vi "FindMutationByVerIndex.vi"(6 "SerializedClassName":string, 7 "default object":refnum<class "BlueSerializable.lvclass">, 8 "error in (no error)":errorcluster, 9 "Old Name Index":u8, 10 "Library Version":T3, 11 "Mutation History":T4 {"LabVIEW Version" format="%.0x"}) -> (0 "error out":errorcluster, 1 "BlueSerializableVersion":T1, 2 "Mutation Record":T2 {"LabVIEW Version" format="%.0x"})   [LabVIEW 2020, in "BlueSerialization.lvlib" / "BlueSerializer.lvclass"]
uses:
  BlueSerializer.lvclass
  <vilib>/Utility/EditLVLibs/LVClass/Mutation History.ctl
  <vilib>/Utility/EditLVLibs/LVClass/Mutation Record.ctl
  <vilib>/Utility/EditLVLibs/LibVersion.ctl
  BlueSerializableVersion.ctl
  BlueSerializable/BlueSerializable.lvclass
  <resource>/Framework/Providers/BlueSerializationProviderShared/UserCommentToVersion.vi
  <vilib>/Utility/error.llb/Error Cluster From Error Code.vi
  <vilib>/ErrorRing/Error Ring.xnode
  BlueSerializer.lvclass/BlueSerializer.ctl
  <resource>/Framework/Providers/BlueSerializationProviderShared/BlueSerializationProviderShared.lvlib
  <vilib>/Utility/EditLVLibs/Edit LVLibs.lvlib
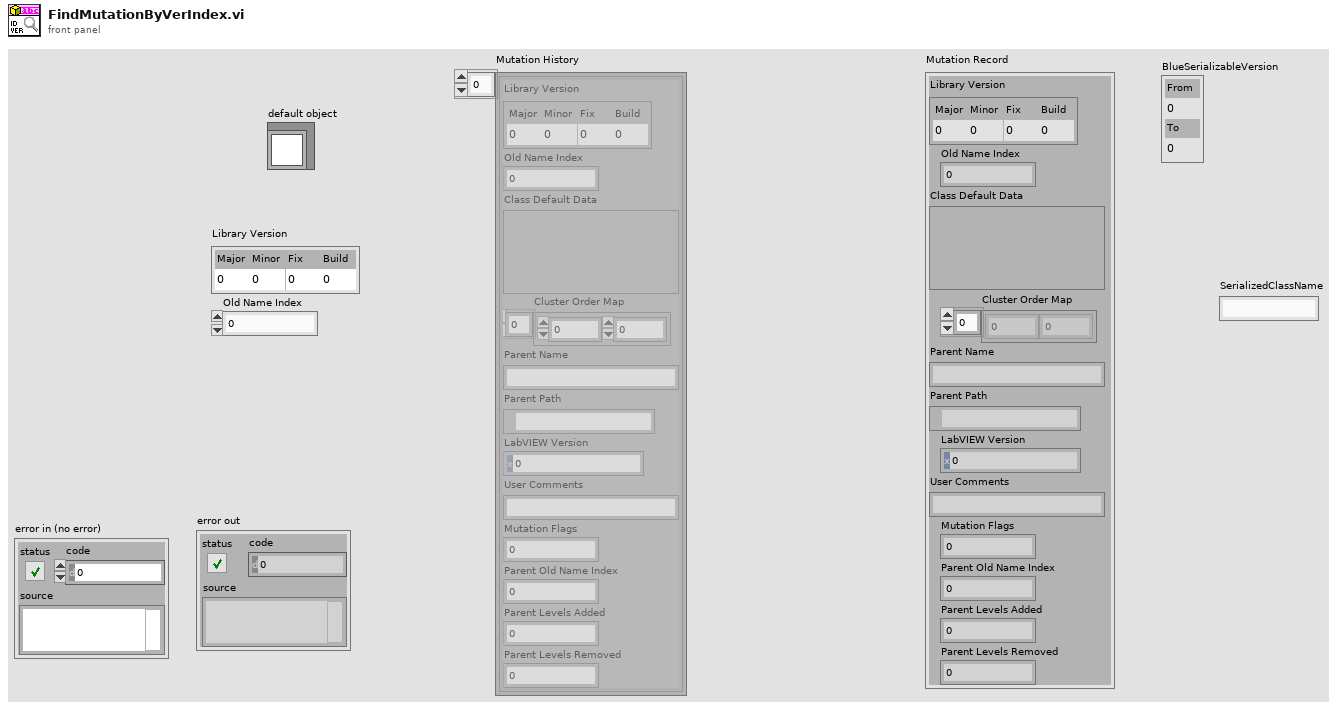
[diagram p1: front panel]
types:
  T1 = typedef "BlueSerialization.lvlib/BlueSerializer.lvclass/BlueSerializableVersion.ctl" = cluster{"From":u16, "To":u16}
  T2 = typedef "Edit LVLibs.lvlib/Mutation Record.ctl" = cluster{"Library Version":T3, "Old Name Index":u8, "Class Default Data":variant, "Cluster Order Map":u32[], "Parent Name":string, "Parent Path":path, "LabVIEW Version":u32, "User Comments":string, "Mutation Flags":u8, "Parent Old Name Index":u8, "Parent Levels Added":u16, "Parent Levels Removed":u16}
  T3 = typedef "Edit LVLibs.lvlib/LibVersion.ctl" = cluster{"Major":u16, "Minor":u16, "Fix":u16, "Build":u16}
  T4 = typedef "Edit LVLibs.lvlib/Mutation History.ctl" = T2[]
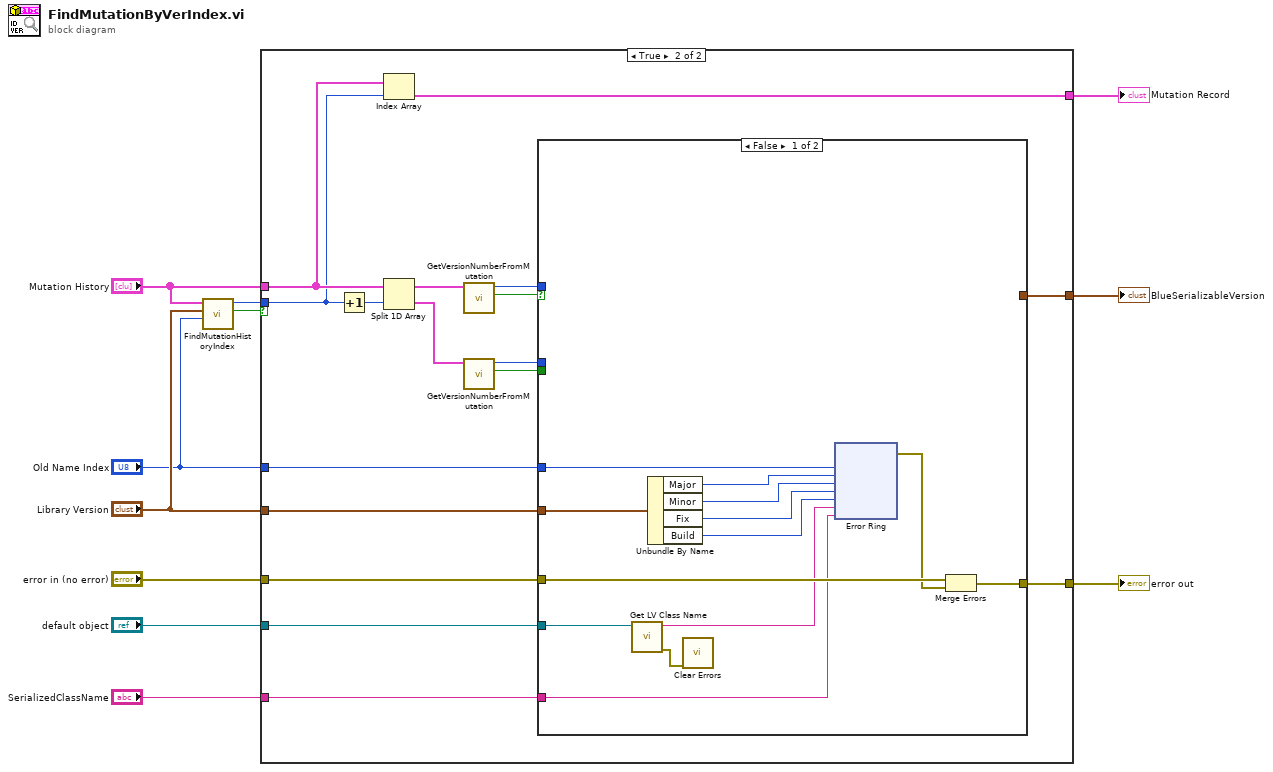
[diagram p0: block diagram]
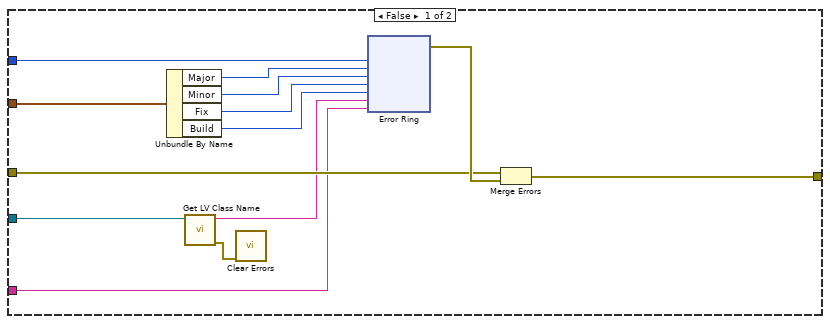
[diagram p2: hidden frame]
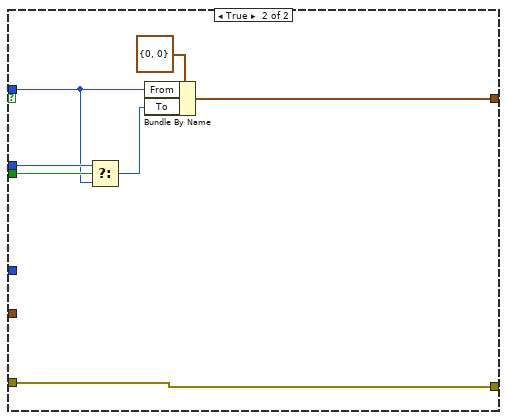
[diagram p3: hidden frame]
diagram:
  n1 = call <resource>:"FindMutationHistoryIndex.vi"("Old Name Index"="Old Name Index", "Library Version"="Library Version", "Mutation History"="Mutation History") -> ("Found?"=w5:bool, "Index"=w6:i32)  [unwired: 7 in]
  n2 = case shown="True" w5 {
    tunnel: "Library Version" -> [w24 w52]
    tunnel: "error in (no error)" -> [w18 w51]
    tunnel: [w17 w50] -> w10
    tunnel: w6 -> [_ w48]
    tunnel: "Mutation History" -> [_ w53]
    tunnel: [_ w54] -> w9
    tunnel: [_ w49] -> w8
    tunnel: "Old Name Index" -> [w16 w40]
    tunnel: "default object" -> [w15 w39]
    tunnel: "SerializedClassName" -> [w12 w38]
    frame False {
      n3 = Unbundle By Name(w24) -> ("Major"=w23:u16, "Minor"=w22:u16, "Fix"=w21:u16, "Build"=w20:u16)
      n4 = call <vilib>:"Get LV Class Name.vi"("object"=w15) -> ("error out"=w13:errorcluster, "class name"=w14:string)  [unwired: 9 in]
      n5 = call <vilib>:"Clear Errors.vi"("error in (no error)"=w13) -> ()  [unwired: 5 in, 2 out]
      n6 = xnode "Error Ring"("parameter 0"=w16, "parameter 1"=w23, "parameter 2"=w22, "parameter 3"=w21, "parameter 4"=w20, "parameter 5"=w14, "parameter 6"=w12) -> ("error out"=w19:errorcluster)
      n7 = Merge Errors(w18, w19) -> (w17:errorcluster)
    }
    frame True {
      n8 = Increment(x=w48) -> (x+1=w47:i32)
      n9 = Index Array(array=w53, index=w48) -> (element=w54:T2)
      n10 = Split 1D Array(array=w53, index=w47) -> (first subarray=w46:T4, second subarray=w41:T4)
      n11 = call <resource>:"GetVersionNumberFromMutation.vi"("Mutation History"=w46) -> ("BlueSerializableVersion found?"=w44:bool, "BlueSerializableVersion"=w45:u16)  [unwired: 9 in]
      n12 = call <resource>:"GetVersionNumberFromMutation.vi"("Mutation History"=w41) -> ("BlueSerializableVersion found?"=w42:bool, "BlueSerializableVersion"=w43:u16)  [unwired: 9 in]
      n13 = case shown="False" w44 {
        tunnel: w42 -> [_ w86]
        tunnel: w45 -> [_ w84]
        tunnel: w43 -> [_ w85]
        tunnel: w52 -> [w63 _]
        tunnel: w51 -> [w62 w82]
        tunnel: [w60 w82] -> w50
        tunnel: [_ w81] -> w49
        tunnel: w40 -> [w59 _]
        tunnel: w39 -> [w57 _]
        tunnel: w38 -> [w55 _]
        frame False {
          n14 = call <vilib>:"Get LV Class Name.vi"("object"=w57) -> ("error out"=w58:errorcluster, "class name"=w56:string)  [unwired: 9 in]
          n15 = Unbundle By Name(w63) -> ("Major"=w67:u16, "Minor"=w66:u16, "Fix"=w65:u16, "Build"=w64:u16)
          n16 = call <vilib>:"Clear Errors.vi"("error in (no error)"=w58) -> ()  [unwired: 5 in, 2 out]
          n17 = xnode "Error Ring"("parameter 0"=w59, "parameter 1"=w67, "parameter 2"=w66, "parameter 3"=w65, "parameter 4"=w64, "parameter 5"=w56, "parameter 6"=w55) -> ("error out"=w61:errorcluster)
          n18 = Merge Errors(w62, w61) -> (w60:errorcluster)
        }
        frame True {
          n19 = Select(t=w85, s=w86, f=w84) -> (s? t:f=w83:u16)
          n20 = Bundle By Name(cluster=T1 {"From"=0, "To"=0} ("Cluster"), "From"=w84, "To"=w83) -> (w81:T1)
        }
      }
    }
  }
  "Mutation Record" <- w9
  "error out" <- w10
  "BlueSerializableVersion" <- w8
